vi "Handle Command.vi"(8 "error in (no error)":errorcluster, 9 "Data":variant, 10 "Command":string, 11 "Instrument.Lockin":refnum<class "Instrument.Lockin.lvclass">) -> (0 "error out":errorcluster, 1 "Processed Data":variant, 2 "Command":string, 3 "Instrument.Lockin out":refnum<class "Instrument.Lockin.lvclass">)   [LabVIEW 2019, in "Instrument.Lockin.lvlib" / "Instrument.Lockin.lvclass"]
uses:
  Instrument.Lockin.lvclass
  Typedefs/API/Lockin.Commands.Local--Enum.ctl
  Typedefs/API/Lockin.Commands--Enum.ctl
  Instrument.Lockin.lvclass/Instrument.Lockin.ctl
  <userlib>/LevyLab/Instrument Framework/Instrument Types/Lockin/Typedefs/LockinAPI.Sampling.Sampling--Cluster.ctl
  <userlib>/LevyLab/Instrument Framework/Instrument Types/Lockin/Typedefs/LockinAPI.Sampling.FsMode--enum.ctl
  <userlib>/LevyLab/Instrument Framework/Instrument Types/Lockin/Typedefs/LockinAPI.getState.states--enum.ctl
  <userlib>/LevyLab/Instrument Framework/Instrument Types/Lockin/Typedefs/LockinAPI.SweepData--Cluster.ctl
  Typedefs/API/Lockin.setState--cluster.ctl
  Instrument.DAQ/Typedefs/State--enum.ctl
  Typedefs/API/Lockin.setLogMode--cluster.ctl
  Typedefs/API/Lockin.setAO_Amp--cluster.ctl
  Typedefs/API/Lockin.setAO_DC--cluster.ctl
  Typedefs/API/Lockin.setAO_f--cluster.ctl
  Typedefs/API/Lockin.setAO_phi--cluster.ctl
  Typedefs/API/Lockin.setAO_function--cluster.ctl
  Instrument.DAQ/Typedefs/AO.Channel.Function--Enum.ctl
  Instrument.DAQ/Typedefs/AO.Channel--Cluster--Array.ctl
  Instrument.DAQ/Typedefs/AO.Channel--Cluster.ctl
  Typedefs/API/Lockin.setREF_f--cluster.ctl
  Typedefs/REF Parameter--Enum.ctl
  Typedefs/API/Lockin.setREF_phi--cluster.ctl
  Typedefs/API/Lockin.setREF_TC--cluster.ctl
  Typedefs/API/Lockin.setREF_RollOff--cluster.ctl
  Instrument.DAQ/Typedefs/REF.Channel--Cluster--Array.ctl
  Instrument.DAQ/Typedefs/REF.Channel--Cluster.ctl
  Instrument.DAQ/Typedefs/Sweep.Configuration--Cluster.ctl
  Instrument.DAQ/Typedefs/Sweep.Channel--Cluster--Array.ctl
  Instrument.DAQ/Typedefs/Sweep.Channel--Cluster.ctl
  Instrument.DAQ/Typedefs/Sweep.Pattern--Enum.ctl
  Typedefs/API/Lockin.setSweep_Time--cluster.ctl
  Typedefs/API/Lockin.setSweep_Table--cluster.ctl
  Instrument.DAQ/Typedefs/DAQ.Sampling.Sampling--Cluster.ctl
  Typedefs/API/Lockin.setSamplingFsMode--cluster.ctl
  Instrument.DAQ/Typedefs/DAQ.Sampling.Fs Mode--enum.ctl
  Instrument.DAQ/Typedefs/Channel.Gain--Cluster.ctl
  Instrument.DAQ/Typedefs/DAQ.Configuration--Cluster--Array.ctl
  Instrument.DAQ/Typedefs/DAQ.Configuration--Cluster.ctl
  Instrument.DAQ/Typedefs/DAQ.Config.AO.Range--enum.ctl
  Instrument.DAQ/Typedefs/DAQ.TerminalConfiguration--ring.ctl
  Instrument.DAQ/Typedefs/DAQ.Config.AI.Range--enum.ctl
  Instrument.DAQ/Typedefs/DAQ.Config.AI.Coupling--enum.ctl
  Instrument.DAQ/Typedefs/PrivateEvents--DAQ.showUI.ctl
  Instrument.DAQ/Typedefs/AI.Channel--Cluster--Array.ctl
  Instrument.DAQ/Typedefs/AI.Channel--Cluster.ctl
  Instrument.DAQ/Typedefs/Simulation Mode--enum.ctl
  Typedefs/Offset Mode--Enum.ctl
  Instrument.DAQ/Typedefs/PrivateEvents--DAQ.setCalibration.ctl
  Instrument.DAQ/Typedefs/Configuration.Prefilter--Cluster.ctl
  Instrument.DAQ/Typedefs/Configuration.LinkFrequencies--Cluster.ctl
  Instrument.DAQ/Typedefs/Configuration.AmplitudeLimit--Cluster.ctl
  Instrument.DAQ/Typedefs/Configuration.DCLimit--Cluster.ctl
  Instrument.DAQ/Typedefs/Configuration.DutyCycle--Cluster.ctl
  Typedefs/API/Lockin.setSamplingMode--cluster.ctl
  Instrument.DAQ/Typedefs/DAQ.Sampling.Sample Mode--Ring.ctl
  afc408c1-4a47-494c-817e-7b9f9bb33729.vi
  a7ccf487-04bf-437f-bc58-012293c091eb.vi
  06f5bff1-b823-416c-a758-fc672ecfcc99.vi
  029a7bc4-99e9-4f65-b437-c26585c9cd40.vi
  95117756-58c8-4cf5-b4a1-eea4f9571e2f.vi
  d527b0ad-2cbe-40d7-81d2-49d8d0078832.vi
  c6561379-f98d-4793-93aa-fc4f7b6fa2da.vi
  f7b28b50-f868-4d06-8d90-790d331e6843.vi
  3b890341-4124-4342-9d75-403cba162ea7.vi
  efd52b93-d691-4a9b-b54f-f4c6778ec2a4.vi
  1b48001d-6f4c-40ce-9883-2cfdfc5b0066.vi
  2465c698-e437-4a4f-8860-a626a4e5f6de.vi
  451a16e7-7f0f-4872-98b2-f896a68061ac.vi
  ce862ac6-3818-4682-989c-38fcf43d7c0a.vi
  0f1e83ab-c55c-46b9-bca3-9d617c6a026d.vi
  c46d61d8-ad78-4a4f-bd83-bba7d42c3393.vi
  06811b67-d74b-4972-af3b-9250fa170671.vi
  148daf87-aacf-4ea0-9f45-6b19ec731a12.vi
  b666889e-e9d3-40fa-bff7-b740bef29075.vi
  7fa0c9c7-d96f-42eb-b083-8fec20da1e25.vi
  2eef0b96-7480-46b2-a416-598848f5f946.vi
  4baefe16-dd55-4900-a34f-f85402a43af0.vi
  bf5afc16-6b2f-47bd-9035-54b404507785.vi
  df248ea2-cdbc-4a64-a66c-167358fcc18f.vi
  f4b2f717-a3e3-4701-aa1a-36f1ad587562.vi
  cb03029c-6dea-422e-9ff0-c01ba24202a7.vi
  ea7ae40a-427f-4df9-8330-54c2df2a5be0.vi
  d5077292-e533-4b52-a4d7-ebb5f6280e78.vi
  be7fa38f-04e0-4644-9c08-a6c1d8484273.vi
  228c5f99-5a8a-4ac9-8c3f-6c80f04cbb43.vi
  29174cef-b5b4-4b3d-8dd9-d067235044c7.vi
  0557ee3d-f7cd-4618-85ce-94304b7e905c.vi
  d91f965c-decf-4ad0-9779-3bd2f4599088.vi
  d9adaec0-ad08-4a9e-8669-6c491ae292cb.vi
  acd43294-18b9-4ae6-b527-f08772f90be2.vi
  6a1e6d83-5b10-4acb-978a-0f1ae3d31a35.vi
  847e6f07-fde4-45b3-9907-c341240c9864.vi
  b8b9aa39-8fbe-4465-abb6-4b3c602a596b.vi
  <vilib>/JDP Science/JSONtext/JSON text to Variant.vi
  <vilib>/JDP Science/JSONtext/LVClass Serializer/JSONtext LVClass Serializer.lvclass
  <userlib>/LevyLab/Instrument Framework/Instrument Types/Lockin/Instrument.LockinAPI.lvclass
  Instrument.DAQ/Instrument.DAQ.lvclass
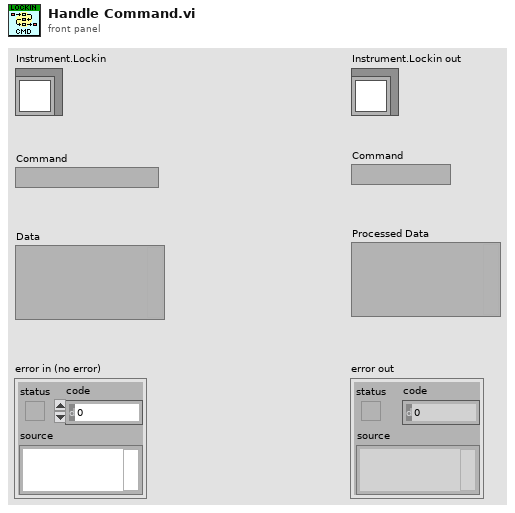
[diagram p1: front panel]
types:
  T1 = typedef "Instrument.Lockin.lvlib/Instrument.Lockin.lvclass/Lockin.Commands.Local--Enum.ctl" = enum16{"autoConfigureDAQ", "setSimulationMode", "zeroPhase", "setCalibration", "setPreFilter", "setFrequencyLink", "setAmplitudeLimit", "setDCLimit", "setDutyCycle", "setSamplingDecimationPreDSP", "setSamplingDecimationPostDSP", "setSamplingMode", "setSamplingFsMultiplier", "setSamplingFsOutput", "setSamplingRefreshRate", "setData_State", "setData_DAQ", "setData_Sampling", "setData_Waveforms", "setData_Results", "setData_SweepWaveforms", "setData_AIChannels", "setData_AOChannels", "setData_REFChannels", "setData_InputGain", "setData_OutputGain", "showUI", "setAI", "setOffset", "setOffsetMode"}
  T2 = typedef "Instrument.Lockin.lvlib/Instrument.Lockin.lvclass/Lockin.Commands--Enum.ctl" = enum16{"setAO", "setAO_Amplitude", "setAO_DC", "setAO_Frequency", "setAO_Phase", "setAO_Function", "setREF", "setREF_Frequency", "setREF_Phase", "setREF_TC", "setREF_Roll-Off", "setDAQ", "setSampling", "setState", "getState", "getAO", "getAI", "getResults", "getSampling", "getAOconfig", "getREFconfig", "setInputGain", "setOutputGain", "getInputGain", "getOutputGain", "setSamplingFsMode", "getSamplingFsMode", "setSweep", "setSweep_Time", "setSweep_Table", "getStatus", "getSweepResults", "getSweepWaveforms", "logConfiguration", "startLogging", "stopLogging"}
  T3 = typedef "Instrument.LockinAPI.lvclass/LockinAPI.Sampling.Sampling--Cluster.ctl" = cluster{"Fs":dbl, "#s":i32}
  T4 = typedef "Instrument.LockinAPI.lvclass/LockinAPI.getState.states--enum.ctl" = enum16{"idle", "created", "started", "stopped", "sweeping"}
  T5 = typedef "Instrument.LockinAPI.lvclass/LockinAPI.SweepData--Cluster.ctl" = cluster{"AO":waveform(dbl)[], "AI":waveform(dbl)[], "X":waveform(dbl)[], "Y":waveform(dbl)[]}
  T6 = cluster{"Time Stamp":timestamp, "Results (Dictionary)":cluster{"key":string, "value":dbl}[]}
  T7 = typedef "Instrument.Lockin.lvlib/Instrument.Lockin.lvclass/Lockin.setState--cluster.ctl" = cluster{"State":T8}
  T8 = typedef "Instrument.Lockin.lvlib/Instrument.DAQ.lvclass/State--enum.ctl" = enum16{"start", "stop", "reset", "start sweep", "stop sweep"}
  T9 = typedef "Instrument.Lockin.lvlib/Instrument.Lockin.lvclass/Lockin.setLogMode--cluster.ctl" = cluster{"interval":u32}
  T10 = enum16{"Amplitude", "DC", "Frequency", "Phase", "Function"}
  T11 = typedef "Instrument.Lockin.lvlib/Instrument.Lockin.lvclass/Lockin.setAO_Amp--cluster.ctl" = cluster{"Channel":i32, "Amplitude":dbl}
  T12 = typedef "Instrument.Lockin.lvlib/Instrument.Lockin.lvclass/Lockin.setAO_DC--cluster.ctl" = cluster{"Channel":i32, "DC":dbl}
  T13 = typedef "Instrument.Lockin.lvlib/Instrument.Lockin.lvclass/Lockin.setAO_f--cluster.ctl" = cluster{"Channel":i32, "Frequency":dbl}
  T14 = typedef "Instrument.Lockin.lvlib/Instrument.Lockin.lvclass/Lockin.setAO_phi--cluster.ctl" = cluster{"Channel":i32, "Phase":dbl}
  T15 = typedef "Instrument.Lockin.lvlib/Instrument.Lockin.lvclass/Lockin.setAO_function--cluster.ctl" = cluster{"Channel":i32, "Function":T16}
  T16 = typedef "Instrument.Lockin.lvlib/Instrument.DAQ.lvclass/AO.Channel.Function--Enum.ctl" = enum16{"sine", "square", "triangle", "saw"}
  T17 = typedef "Instrument.Lockin.lvlib/Instrument.DAQ.lvclass/AO.Channel--Cluster--Array.ctl" = T18[]
  T18 = typedef "Instrument.Lockin.lvlib/Instrument.DAQ.lvclass/AO.Channel--Cluster.ctl" = cluster{"Enable?":bool, "Channel":i32, "Amplitude":dbl, "Offset":dbl, "Frequency":dbl, "Phase":dbl, "Function":T16, "Sweeping?":bool, "Limit AC":bool, "Limit DC?":bool, "Duty Cycle":bool}
  T19 = typedef "Instrument.Lockin.lvlib/Instrument.Lockin.lvclass/Lockin.setREF_f--cluster.ctl" = cluster{"Channel":i32, "Frequency":dbl}
  T20 = typedef "Instrument.Lockin.lvlib/Instrument.Lockin.lvclass/REF Parameter--Enum.ctl" = enum16{"Frequency", "Phase", "Time Constant", "RollOff"}
  T21 = typedef "Instrument.Lockin.lvlib/Instrument.Lockin.lvclass/Lockin.setREF_phi--cluster.ctl" = cluster{"Channel":i32, "Phase":dbl}
  T22 = typedef "Instrument.Lockin.lvlib/Instrument.Lockin.lvclass/Lockin.setREF_TC--cluster.ctl" = cluster{"Channel":i32, "TC":dbl}
  T23 = typedef "Instrument.Lockin.lvlib/Instrument.Lockin.lvclass/Lockin.setREF_RollOff--cluster.ctl" = cluster{"Channel":i32, "Roll-Off":i32}
  T24 = typedef "Instrument.Lockin.lvlib/Instrument.DAQ.lvclass/REF.Channel--Cluster--Array.ctl" = T25[]
  T25 = typedef "Instrument.Lockin.lvlib/Instrument.DAQ.lvclass/REF.Channel--Cluster.ctl" = cluster{"Enable?":bool, "Channel":i32, "Frequency":dbl, "Phase":dbl, "TC":dbl, "Roll-Off":i32}
  T26 = typedef "Instrument.Lockin.lvlib/Instrument.Lockin.lvclass/Lockin.setSweep_Time--cluster.ctl" = cluster{"SweepTime":dbl}
  T27 = typedef "Instrument.Lockin.lvlib/Instrument.Lockin.lvclass/Lockin.setSweep_Table--cluster.ctl" = cluster{"Channel":i32, "Table":dbl[]}
  T28 = typedef "Instrument.Lockin.lvlib/Instrument.DAQ.lvclass/DAQ.Sampling.Sampling--Cluster.ctl" = cluster{"Fs":dbl, "#s":i32}
  T29 = typedef "Instrument.Lockin.lvlib/Instrument.Lockin.lvclass/Lockin.setSamplingFsMode--cluster.ctl" = cluster{"FsMode":T30}
  T30 = typedef "Instrument.Lockin.lvlib/Instrument.DAQ.lvclass/DAQ.Sampling.Fs Mode--enum.ctl" = enum16{"Manual", "Auto Fs", "Max Fs"}
  T31 = typedef "Instrument.Lockin.lvlib/Instrument.DAQ.lvclass/Channel.Gain--Cluster.ctl" = cluster{"Channel":string, "Gain":dbl}
  T32 = typedef "Instrument.Lockin.lvlib/Instrument.DAQ.lvclass/DAQ.Configuration--Cluster--Array.ctl" = T33[]
  T33 = typedef "Instrument.Lockin.lvlib/Instrument.DAQ.lvclass/DAQ.Configuration--Cluster.ctl" = cluster{"Device":string, "Lockin.AO":string, "AO.Ch":string, "AO.Range":T34, "AO terminal config":T35, "Lockin.AI":string, "AI.Ch":string, "AI.Range":T36, "AI.Coupling":T37, "AI terminal config":T35}
  T34 = typedef "Instrument.Lockin.lvlib/Instrument.DAQ.lvclass/DAQ.Config.AO.Range--enum.ctl" = enum16{"±0.1", "±1.0", "±3.5", "±10.0", ""}
  T35 = typedef "Instrument.Lockin.lvlib/Instrument.DAQ.lvclass/DAQ.TerminalConfiguration--ring.ctl" = i32
  T36 = typedef "Instrument.Lockin.lvlib/Instrument.DAQ.lvclass/DAQ.Config.AI.Range--enum.ctl" = enum16{"±0.316", "±1.00", "±3.16", "±10.0", "±31.6", "±42.4", ""}
  T37 = typedef "Instrument.Lockin.lvlib/Instrument.DAQ.lvclass/DAQ.Config.AI.Coupling--enum.ctl" = u16
  T38 = typedef "Instrument.Lockin.lvlib/Instrument.DAQ.lvclass/PrivateEvents--DAQ.showUI.ctl" = bool
  T39 = typedef "Instrument.Lockin.lvlib/Instrument.DAQ.lvclass/AI.Channel--Cluster--Array.ctl" = T40[]
  T40 = typedef "Instrument.Lockin.lvlib/Instrument.DAQ.lvclass/AI.Channel--Cluster.ctl" = cluster{"Enable?":bool, "Channel":i32, "References":u16[], "reference index":i32}
  T41 = typedef "Instrument.Lockin.lvlib/Instrument.DAQ.lvclass/Simulation Mode--enum.ctl" = enum16{"AI = HW simulated", "AI = noise*AO", "AI = waveguide"}
  T42 = typedef "Instrument.Lockin.lvlib/Instrument.Lockin.lvclass/Offset Mode--Enum.ctl" = enum16{"Measure", "Remove"}
  T43 = typedef "Instrument.Lockin.lvlib/Instrument.DAQ.lvclass/PrivateEvents--DAQ.setCalibration.ctl" = enum16{"Check", "Calibrate"}
  T44 = typedef "Instrument.Lockin.lvlib/Instrument.DAQ.lvclass/Configuration.Prefilter--Cluster.ctl" = cluster{"60 Hz":bool, "Low Pass":bool, "Low Pass Cutoff (Hz)":dbl}
  T45 = typedef "Instrument.Lockin.lvlib/Instrument.DAQ.lvclass/Configuration.LinkFrequencies--Cluster.ctl" = cluster{"Link?":bool, "Frequency (Hz)":dbl}
  T46 = typedef "Instrument.Lockin.lvlib/Instrument.DAQ.lvclass/Configuration.DCLimit--Cluster.ctl" = cluster{"Limit?":bool, "Limit (V)":dbl}
  T47 = typedef "Instrument.Lockin.lvlib/Instrument.DAQ.lvclass/Configuration.DutyCycle--Cluster.ctl" = cluster{"Option?":bool, "Duty Cycle (%)":dbl}
  T48 = typedef "Instrument.Lockin.lvlib/Instrument.Lockin.lvclass/Lockin.setSamplingMode--cluster.ctl" = cluster{"SampleMode":T49}
  T49 = typedef "Instrument.Lockin.lvlib/Instrument.DAQ.lvclass/DAQ.Sampling.Sample Mode--Ring.ctl" = i32
  T50 = typedef "Instrument.LockinAPI.lvclass/LockinAPI.Sampling.FsMode--enum.ctl" = enum16{"Manual", "Auto Fs", "Max Fs"}
  T51 = typedef "Instrument.Lockin.lvlib/Instrument.DAQ.lvclass/Status--enum.ctl" = enum16{"idle", "created", "started", "stopped", "sweeping"}
  T52 = typedef "Instrument.Lockin.lvlib/Instrument.DAQ.lvclass/Channel.Gain--Cluster--Array.ctl" = T31[]
  T53 = typedef "Instrument.Lockin.lvlib/Instrument.DAQ.lvclass/Results--Cluster.ctl" = cluster{"Time Stamp":timestamp, "Results (Dictionary)":cluster{"key":string, "value":dbl[]}[]}
  T54 = typedef "Instrument.Lockin.lvlib/Instrument.DAQ.lvclass/Sweep.Configuration--Cluster.ctl" = cluster{"sweepTime":dbl, "initialWaitTime":dbl, "returnToStart":bool, "sweepChannels":T55}
  T55 = typedef "Instrument.Lockin.lvlib/Instrument.DAQ.lvclass/Sweep.Channel--Cluster--Array.ctl" = T56[]
  T56 = typedef "Instrument.Lockin.lvlib/Instrument.DAQ.lvclass/Sweep.Channel--Cluster.ctl" = cluster{"Enable?":bool, "Channel":u16, "Start":dbl, "End":dbl, "Pattern":T57, "Table":dbl[]}
  T57 = typedef "Instrument.Lockin.lvlib/Instrument.DAQ.lvclass/Sweep.Pattern--Enum.ctl" = enum16{"Ramp /", "Ramp /\\", "Smooth Ramp _/", "Smooth Ramp _/\\_", "Table"}
  T58 = typedef "Instrument.Lockin.lvlib/Instrument.DAQ.lvclass/DAQ.Sampling--Cluster.ctl" = cluster{"Sampling":T28, "sample mode":i32, "Fs Mode":T30, "Fs Multiplier":dbl, "Refresh Rate (Hz)":dbl, "Decimation.PreDSP":i32, "Decimation.PostDSP":i32, "Fs.Output":dbl}
  T59 = typedef "Instrument.Lockin.lvlib/Instrument.DAQ.lvclass/DAQ.Config.AO--Cluster--Array.ctl" = cluster{"Channels":tag, "Range":T34, "terminal configuration":T35, "Type":T60}[]
  T60 = typedef "Instrument.Lockin.lvlib/Instrument.DAQ.lvclass/DAQ.Type--enum.ctl" = enum16{"None", "USB-4431", "PXI-446x"}
  T61 = typedef "Instrument.Lockin.lvlib/Instrument.DAQ.lvclass/DAQ.Config.AI--Cluster--Array.ctl" = cluster{"Channels":tag, "Coupling":T37, "Range":T36, "terminal configuration":T35, "Type":T60}[]
  T62 = typedef "Instrument.Lockin.lvlib/Instrument.DAQ.lvclass/PublicEvents--DAQ.getWaveforms.ctl" = cluster{"AO":waveform(dbl)[], "AI":waveform(dbl)[], "REF_X":waveform(dbl)[], "REF_Y":waveform(dbl)[], "X":waveform(dbl)[], "Y":waveform(dbl)[]}
  T63 = typedef "Instrument.Lockin.lvlib/Instrument.DAQ.lvclass/PublicEvents--DAQ.getSweepWaveforms.ctl" = cluster{"AO":waveform(dbl)[], "AI":waveform(dbl)[], "X":waveform(dbl)[], "Y":waveform(dbl)[]}
  T64 = typedef "Instrument.Lockin.lvlib/Instrument.DAQ.lvclass/Configuration.AmplitudeLimit--Cluster.ctl" = cluster{"Limit?":bool, "Limit (V)":dbl}
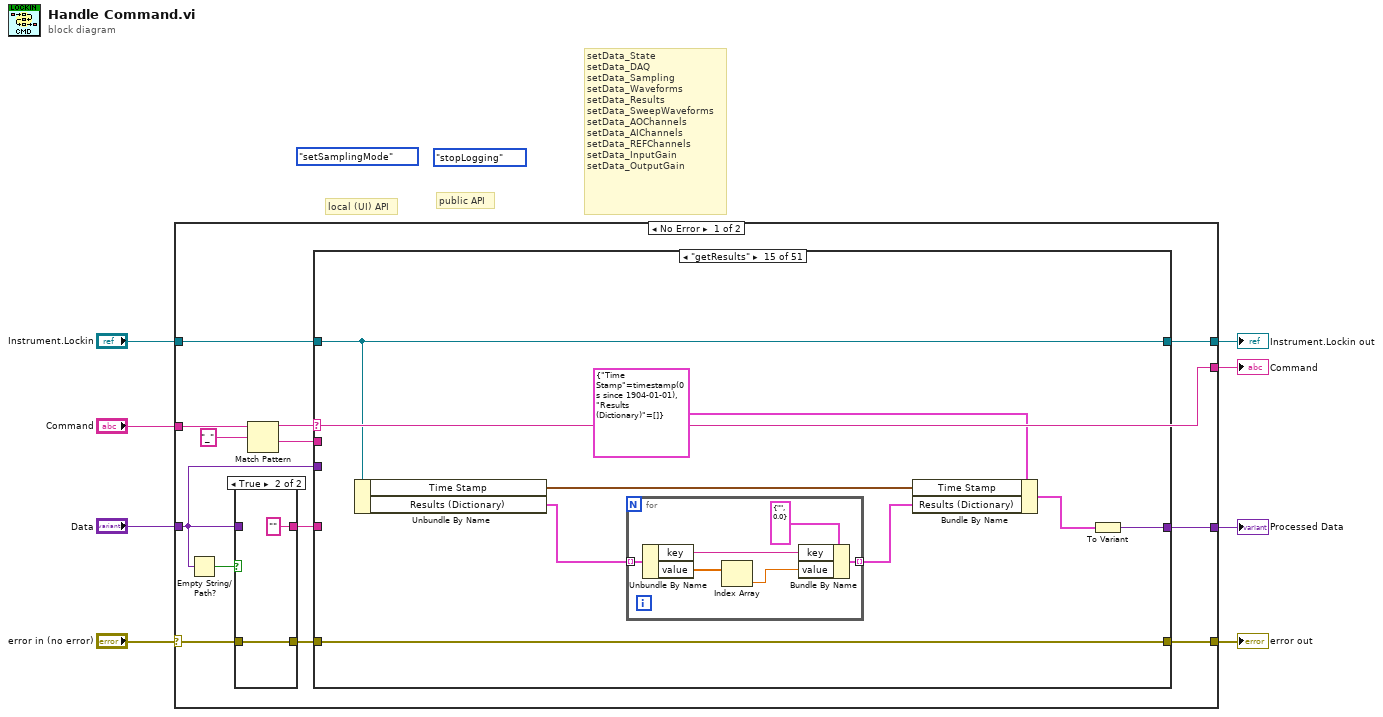
[diagram p0: block diagram]
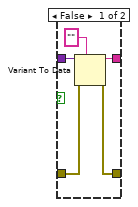
[diagram p2: hidden frame]
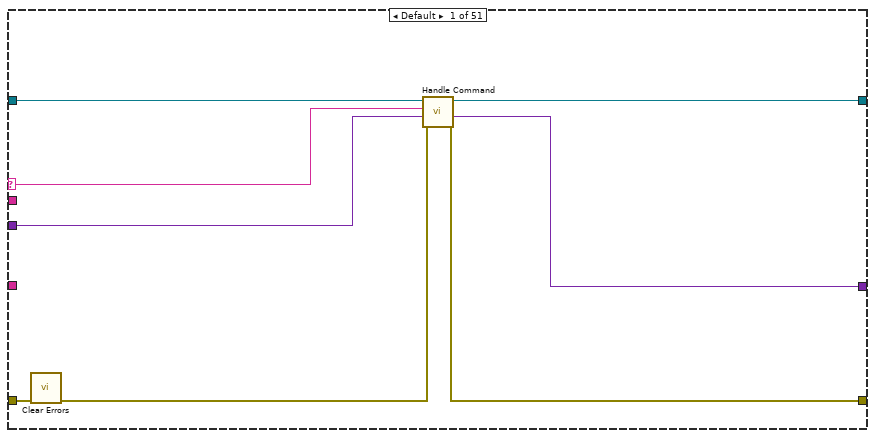
[diagram p3: hidden frame]
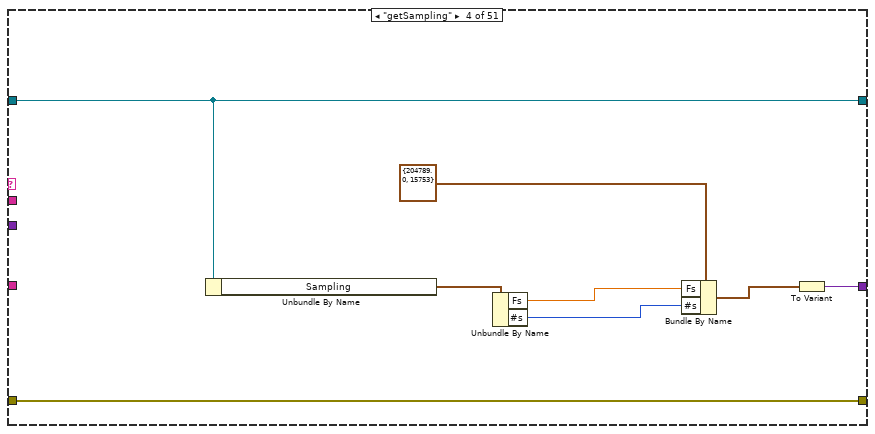
[diagram p6: hidden frame]
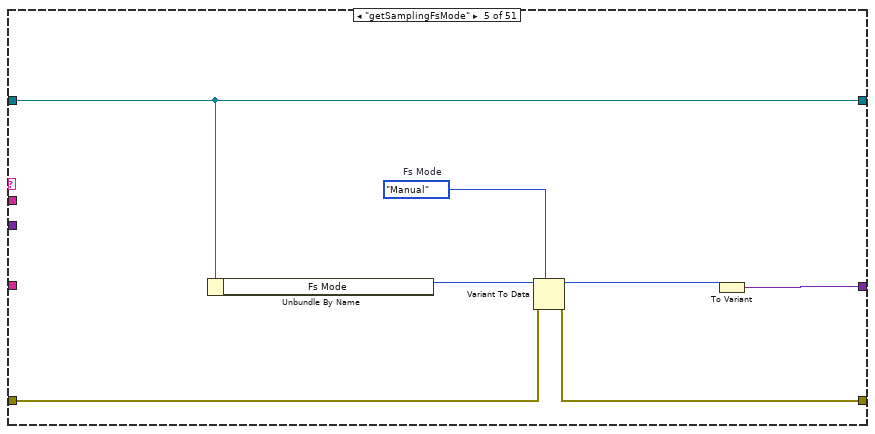
[diagram p7: hidden frame]
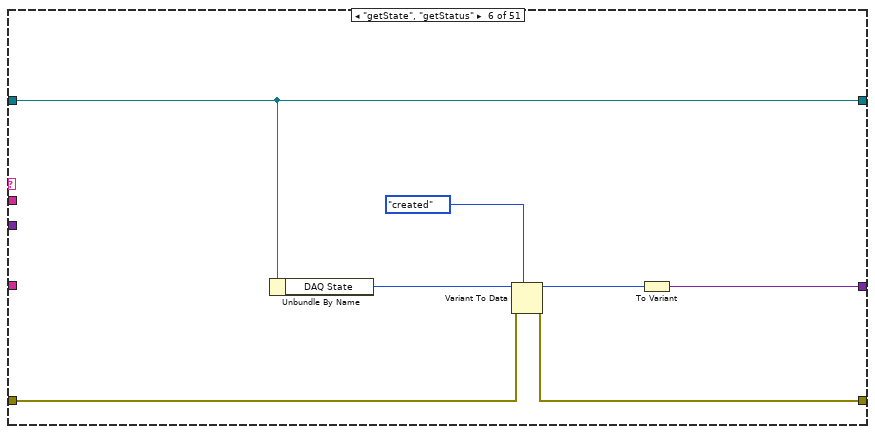
[diagram p8: hidden frame]
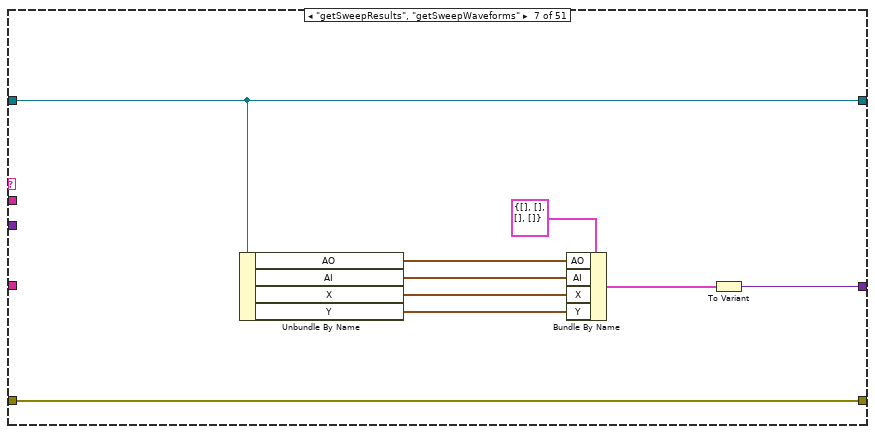
[diagram p9: hidden frame]
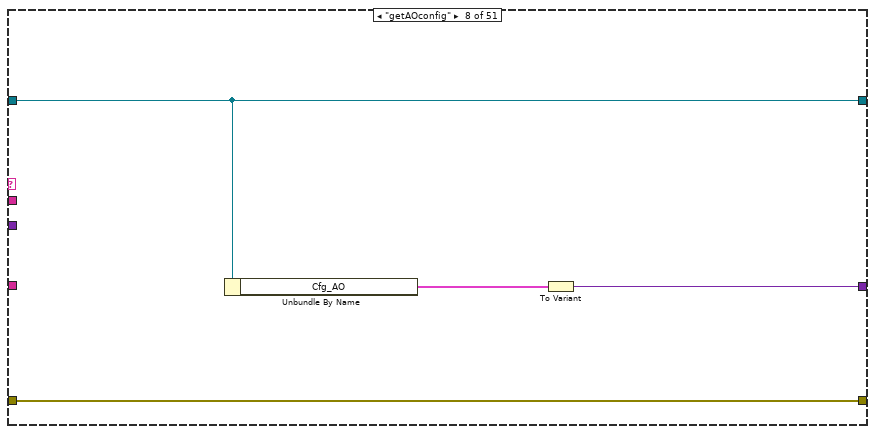
[diagram p10: hidden frame]
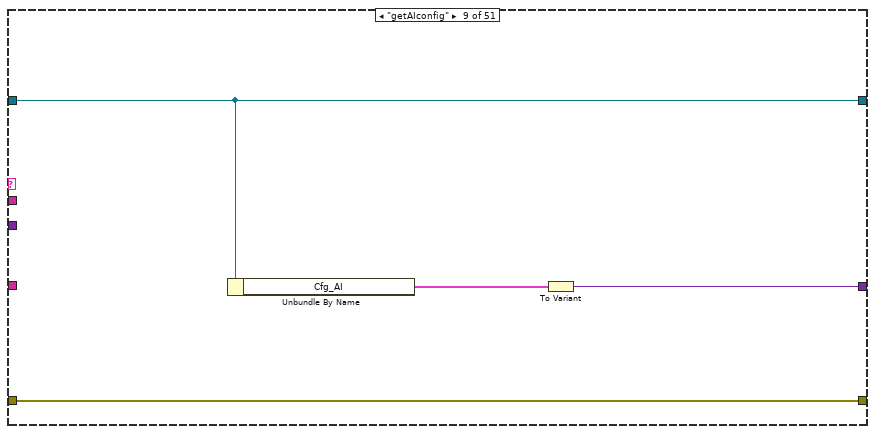
[diagram p11: hidden frame]
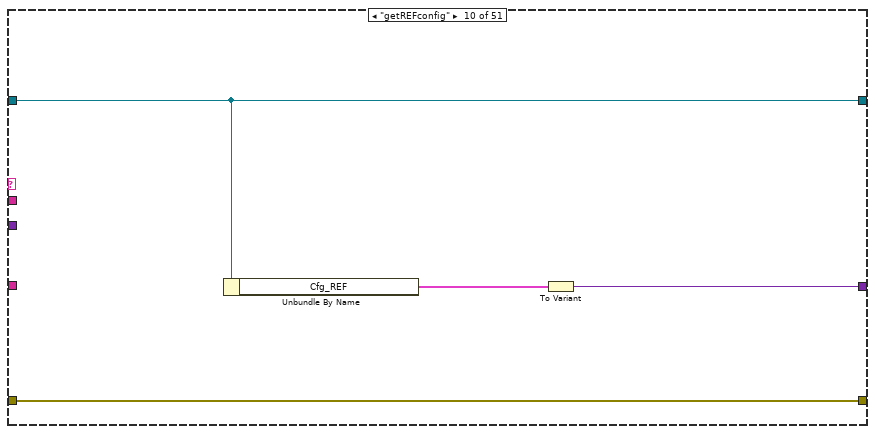
[diagram p12: hidden frame]
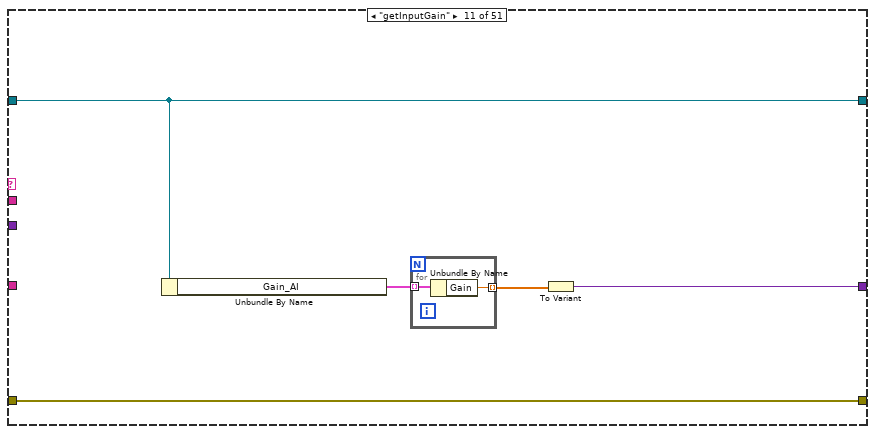
[diagram p13: hidden frame]
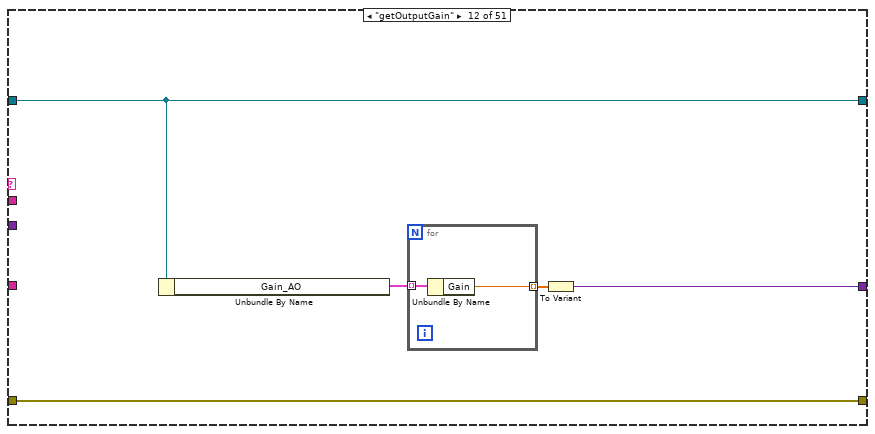
[diagram p14: hidden frame]
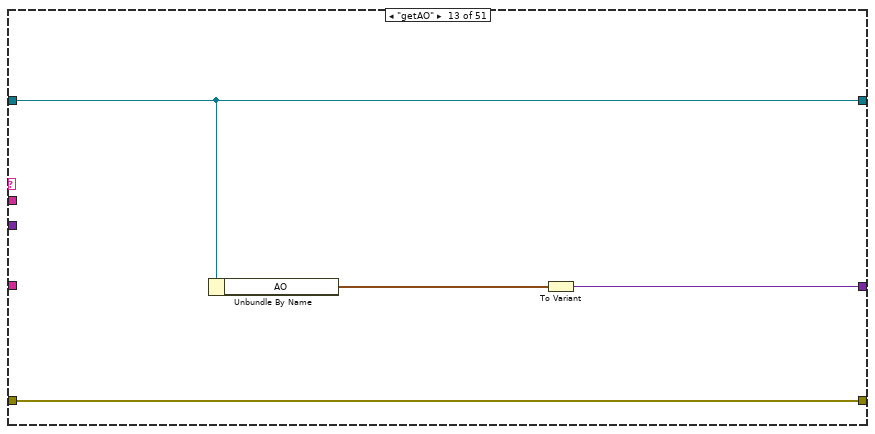
[diagram p15: hidden frame]
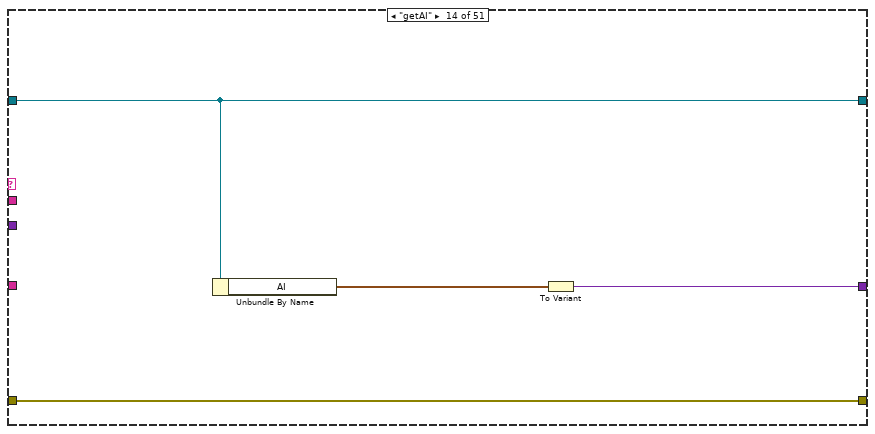
[diagram p16: hidden frame]
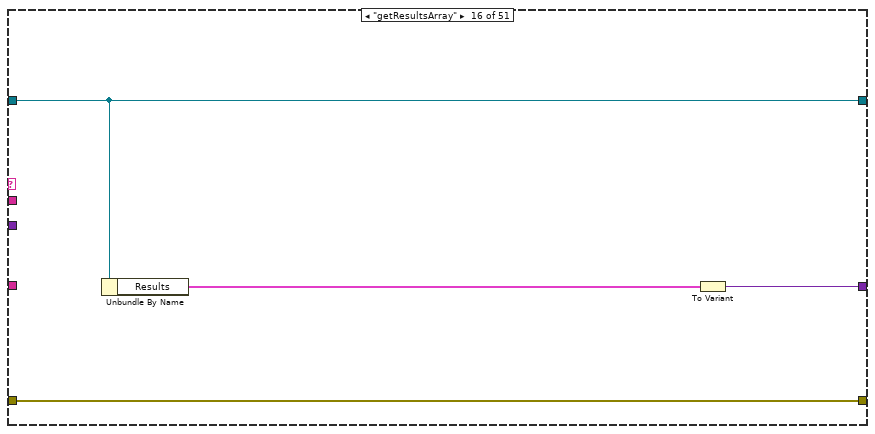
[diagram p17: hidden frame]
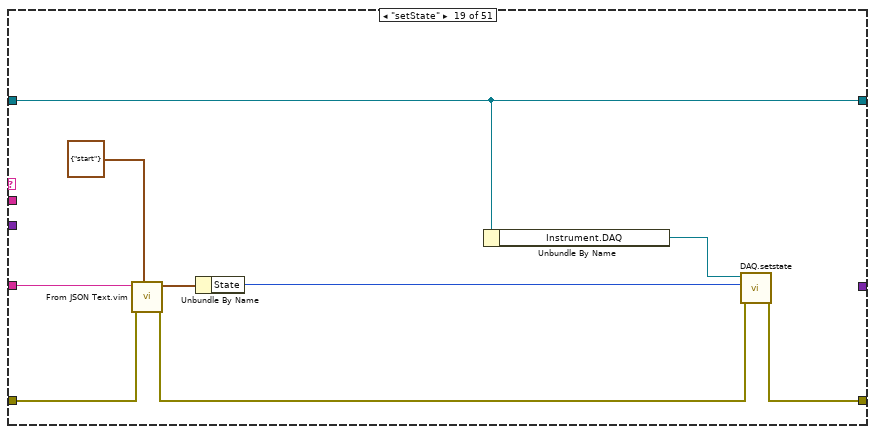
[diagram p20: hidden frame]
diagram:
  (unwired) Lockin.Commands.Local--Enum."setSamplingMode" ("Enum")
  (unwired) Lockin.Commands--Enum."stopLogging" ("Enum")
  # "setData_State\nsetData_DAQ\nsetData_Sampling\nsetData_Waveforms\nsetData_Results\nsetData_SweepWaveforms\nsetData_AOChannels\nsetData_AIChannels\nsetData_REFChannels\nsetData_InputGain\nsetData_OutputGain"
  # "local (UI) API"
  # "public API"
  n1 = case shown="No Error" "error in (no error)" {
    selector: "error in (no error)" -> [w17 w708]
    tunnel: [w18 w708] -> w7
    tunnel: [w20 w707] -> w6
    tunnel: "Instrument.Lockin" -> [w21 w707]
    tunnel: "Command" -> [w12 w706]
    tunnel: [w19 variant] -> w5
    tunnel: "Data" -> [w9 _]
    tunnel: [w11 w706] -> w3
    frame No Error {
      n2 = Empty String/Path?(string/path=w9) -> (empty?=w10:bool)
      n3 = case shown="True" w10 {
        tunnel: w17 -> [w26 w27]
        tunnel: [w24 ""] -> w16
        tunnel: [w23 w27] -> w13
        tunnel: w9 -> [w22 _]
        frame False {
          n4 = Variant To Data(error in=w26, type="", Variant=w22) -> (data=w24:string, error out=w23:errorcluster)
        }
        frame True {
        }
      }
      n5 = Match Pattern(string=w12, regular expression="_") -> (before substring=w11:string, after substring=w14:string)  [unwired: 1 in, 2 out]
      n6 = case shown="\"getResults\"" w11 {
        selector: w11 -> [w31 _ _ _ _ _ _ _ _ _ _ _ _ _ _ _ _ _ _ _ _ _ _ _ _ _ _ _ _ _ _ _ _ _ _ _ _ _ _ _ _ _ _ _ _ _ _ _ _ _ _]
        tunnel: w21 -> [w36 w38 w40 w46 w54 w61 w69 w72 w76 w80 w86 w93 w98 w102 w111 w121 w125 w127 w131 w140 w147 w151 w156 w230 w293 w325 w340 w349 w367 w386 w403 w414 w416 w430 w438 w552 w565 w575 w585 w593 w600 w612 w622 w632 w642 w650 w660 w674 w684 w694 w704]
        tunnel: [w34 w38 w40 w46 w54 w61 w69 w72 w76 w80 w86 w93 w98 w102 w111 w121 w125 w127 w131 w140 w147 w151 w154 w225 w297 w324 w337 w350 w368 w387 w402 w414 w416 w424 w434 w552 w564 w575 w585 w593 w601 w613 w623 w633 w643 w649 w659 w671 w681 w691 w701] -> w20
        tunnel: [w35 _ _ w48 w55 w62 w71 w74 w78 w82 w88 w95 w101 w105 w113 w123 _ _ _ _ _ _ _ _ _ _ _ _ _ _ _ _ _ _ _ _ _ w566 _ _ _ _ _ _ _ _ _ _ _ _ _] -> w19
        tunnel: w16 -> [_ _ _ _ _ _ _ _ _ _ _ _ _ _ _ _ _ _ w136 w144 _ _ w160 w233 w301 w331 w342 w355 w373 w391 w412 _ w422 w432 w436 _ w559 w572 _ w590 w597 w608 w618 w631 w641 w648 w658 w669 w678 w688 w699]
        tunnel: [w32 w37 w39 w47 w50 w57 w70 w73 w77 w81 w87 w94 w100 w104 w112 w122 w124 w126 w132 w137 w146 w150 w157 w226 w298 w327 w335 w351 w369 w388 w407 w413 w417 w426 w433 w554 w560 w573 w583 w591 w602 w609 w619 w625 w634 w651 w661 w670 w680 w690 w700] -> w18
        tunnel: w14 -> [_ _ _ _ _ _ _ _ _ _ _ _ _ _ _ _ _ _ _ _ _ _ w155 w231 w294 _ _ _ _ _ _ _ _ _ w437 _ _ _ _ _ _ _ _ _ _ _ _ _ _ _ _]
        tunnel: w13 -> [w33 w37 w39 w47 w49 w56 w70 w73 w77 w81 w87 w94 w100 w104 w112 w122 w124 w126 w135 w143 w145 w148 w159 w232 w300 w329 w341 w354 w372 w390 w411 w413 w419 w431 w435 w553 w558 w569 w584 w586 w595 w606 w615 w629 w639 w647 w657 w668 w676 w687 w696]
        tunnel: w9 -> [w30 _ _ _ _ _ _ _ _ _ _ _ _ _ _ _ _ _ _ _ _ _ _ _ _ _ _ _ _ _ _ _ _ _ _ _ _ _ _ _ _ _ _ _ _ _ _ _ _ _ _]
        frame Default {
          n7 = call <vilib>:"Clear Errors.vi"("error in (no error)"=w33) -> ("error out"=w29:errorcluster)  [unwired: 5 in, 1 out]
          n8 = call-parent "Handle Command.vi"("error in (no error)"=w29, "params in"=w30, "command"=w31, "Instrument in"=w36) -> ("error out"=w32:errorcluster, "processed data"=w35:variant, "Instrument out"=w34:refnum<class "Instrument.Lockin.lvclass">)  [unwired: 4 in, 1 out]
        }
        frame "----------PUBLIC API----------" {
        }
        frame "----------GET METHODS----------" {
        }
        frame "getSampling" {
          n9 = Unbundle By Name(w46) -> ("Sampling"=w44:T28)
          n10 = Unbundle By Name(w44) -> ("Fs"=w43:dbl, "#s"=w42:i32)
          n11 = Bundle By Name(cluster=T3 {"Fs"=204789.0, "#s"=15753} ("sampling"), "Fs"=w43, "#s"=w42) -> (w41:T3)
          n12 = To Variant(anything=w41) -> (Variant=w48:variant)
        }
        frame "getSamplingFsMode" {
          w52 = LockinAPI.Sampling.FsMode--enum."Manual"  # Fs Mode
          n13 = Unbundle By Name(w54) -> ("Fs Mode"=w53:T30)
          n14 = Variant To Data(error in=w49, type=w52, Variant=w53) -> (data=w51:T50, error out=w50:errorcluster)
          n15 = To Variant(anything=w51) -> (Variant=w55:variant)
        }
        frame "getState", "getStatus" {
          n16 = Unbundle By Name(w61) -> ("DAQ State"=w59:T51)
          n17 = Variant To Data(error in=w56, type=LockinAPI.getState.states--enum."created" ("getState.states"), Variant=w59) -> (data=w58:T4, error out=w57:errorcluster)
          n18 = To Variant(anything=w58) -> (Variant=w62:variant)
        }
        frame "getSweepResults", "getSweepWaveforms" {
          n19 = Unbundle By Name(w69) -> ("AO"=w67:waveform(dbl)[], "AI"=w66:waveform(dbl)[], "X"=w65:waveform(dbl)[], "Y"=w64:waveform(dbl)[])
          n20 = Bundle By Name(cluster=T5 {"AO"=[], "AI"=[], "X"=[], "Y"=[]} ("sweepData"), "AO"=w67, "AI"=w66, "X"=w65, "Y"=w64) -> (w63:T5)
          n21 = To Variant(anything=w63) -> (Variant=w71:variant)
        }
        frame "getAOconfig" {
          n22 = Unbundle By Name(w72) -> ("Cfg_AO"=w75:T17)
          n23 = To Variant(anything=w75) -> (Variant=w74:variant)
        }
        frame "getAIconfig" {
          n24 = Unbundle By Name(w76) -> ("Cfg_AI"=w79:T39)
          n25 = To Variant(anything=w79) -> (Variant=w78:variant)
        }
        frame "getREFconfig" {
          n26 = Unbundle By Name(w80) -> ("Cfg_REF"=w83:T24)
          n27 = To Variant(anything=w83) -> (Variant=w82:variant)
        }
        frame "getInputGain" {
          n28 = Unbundle By Name(w86) -> ("Gain_AI"=w85:T52)
          n29 = for {
            tunnel: w85 -> [w90] mode=indexing
            tunnel: [w89] -> w84 mode=indexing
            n30 = Unbundle By Name(w90) -> ("Gain"=w89:dbl)
          }
          n31 = To Variant(anything=w84) -> (Variant=w88:variant)
        }
        frame "getOutputGain" {
          n32 = Unbundle By Name(w93) -> ("Gain_AO"=w92:T52)
          n33 = for {
            tunnel: w92 -> [w97] mode=indexing
            tunnel: [w96] -> w91 mode=indexing
            n34 = Unbundle By Name(w97) -> ("Gain"=w96:dbl)
          }
          n35 = To Variant(anything=w91) -> (Variant=w95:variant)
        }
        frame "getAO" {
          n36 = Unbundle By Name(w98) -> ("AO"=w99:waveform(dbl)[])
          n37 = To Variant(anything=w99) -> (Variant=w101:variant)
        }
        frame "getAI" {
          n38 = Unbundle By Name(w102) -> ("AI"=w103:waveform(dbl)[])
          n39 = To Variant(anything=w103) -> (Variant=w105:variant)
        }
        frame "getResults" {
          n40 = Unbundle By Name(w111) -> ("Time Stamp"=w108:timestamp, "Results (Dictionary)"=w107:cluster{"key":string, "value":dbl[]}[])
          n41 = for {
            tunnel: w107 -> [w118] mode=indexing
            tunnel: [w114] -> w109 mode=indexing
            n42 = Unbundle By Name(w118) -> ("key"=w115:string, "value"=w119:dbl[])
            n43 = Index Array(array=w119) -> (element=w116:dbl)  [unwired: 1 in]
            n44 = Bundle By Name(cluster=cluster{"key":string, "value":dbl} {"key"="", "value"=0.0} ("key-value"), "key"=w115, "value"=w116) -> (w114:cluster{"key":string, "value":dbl})
          }
          n45 = Bundle By Name(cluster=T6 {"Time Stamp"=timestamp(0 s since 1904-01-01), "Results (Dictionary)"=[]} ("input cluster"), "Time Stamp"=w108, "Results (Dictionary)"=w109) -> (w106:T6)
          n46 = To Variant(anything=w106) -> (Variant=w113:variant)
        }
        frame "getResultsArray" {
          n47 = Unbundle By Name(w121) -> ("Results"=w120:T53)
          n48 = To Variant(anything=w120) -> (Variant=w123:variant)
        }
        frame "getAUX" {
        }
        frame "----------SET METHODS----------" {
        }
        frame "setState" {
          n49 = call "From JSON Text.vim"("Data Type and Default Value"=T7 {"State"=enum."start"} ("setState"), "error in (no error)"=w135, "JSON"=w136) -> ("error out"=w133:errorcluster, "Data out"=w129:T7)  [unwired: 7 in]
          n50 = Unbundle By Name(w129) -> ("State"=w128:T8)
          n51 = Unbundle By Name(w131) -> ("Instrument.DAQ"=w134:refnum<class "Instrument.DAQ.lvclass">)
          n52 = call "DAQ.setstate.vi"("error in (no error)"=w133, "setState"=w128, "Instrument.DAQ"=w134) -> ("error out"=w132:errorcluster)  [unwired: 7 in, 1 out]
        }
        frame "startLogging" {
          # "local event API does not need cluster"
          # "remote API store data in cluster"
          n53 = call "From JSON Text.vim"("Data Type and Default Value"=T9 {"interval"=1} ("setLogMode"), "error in (no error)"=w143, "JSON"=w144) -> ("error out"=w138:errorcluster, "Data out"=w142:T9)  [unwired: 7 in]
          n54 = Unbundle By Name(w142) -> ("interval"=w139:u32)
          n55 = call "Lockin.setLogMode.vi"("error in (no error)"=w138, "interval (ms)"=w139, "Instrument.Lockin"=w140) -> ("error out"=w137:errorcluster)  [unwired: 7 in, 1 out]
        }
        frame "logConfiguration" {
          # "local event API does not need cluster"
          # "remote API store data in cluster"
          n56 = call "Lockin.logConfiguration.vi"("error in (no error)"=w145, "Instrument.Lockin"=w147) -> ("error out"=w146:errorcluster)  [unwired: 8 in, 1 out]
        }
        frame "stopLogging" {
          # "local event API does not need cluster"
          n57 = call "Lockin.setLogMode.vi"("error in (no error)"=w148, "interval (ms)"=u32 0 ("interval"), "Instrument.Lockin"=w151) -> ("error out"=w150:errorcluster)  [unwired: 7 in, 1 out]
        }
        frame "setAO" {
          # "Lockin SMO: Set AO"
          # "Adjust Channels"
          n58 = case shown="\"\"" w155 {
            selector: w155 -> [w170 _]
            tunnel: w160 -> [w169 w222]
            tunnel: w159 -> [w168 w221]
            tunnel: [w163 w217] -> w153
            tunnel: w156 -> [w166 w220]
            tunnel: [w167 w219] -> w154
            frame Default {
              n59 = case shown="\"Phase\"" w170 {
                tunnel: w169 -> [w179 w188 w197 w206 w215]
                tunnel: w168 -> [w178 w187 w196 w205 w214]
                tunnel: [w177 w186 w195 w204 w213] -> w164
                tunnel: [T10."Amplitude" ("Parameter") T10."DC" ("Parameter") T10."Frequency" ("Parameter") T10."Phase" ("Parameter") T10."Function" ("Parameter")] -> w165
                tunnel: [w173 w183 w192 w201 w210] -> w162
                tunnel: [w171 w180 w189 w198 w207] -> w161
                frame "Amplitude", Default {
                  n60 = call "From JSON Text.vim"("Data Type and Default Value"=T11 {"Channel"=5, "Amplitude"=0.0} ("setAO_Amp"), "error in (no error)"=w178, "JSON"=w179) -> ("error out"=w177:errorcluster, "Data out"=w175:T11)  [unwired: 7 in]
                  n61 = Unbundle By Name(w175) -> ("Channel"=w173:i32, "Amplitude"=w172:dbl)
                  n62 = To Variant(anything=w172) -> (Variant=w171:variant)
                }
                frame "DC" {
                  n63 = call "From JSON Text.vim"("Data Type and Default Value"=T12 {"Channel"=5, "DC"=0.0} ("setAO_DC"), "error in (no error)"=w187, "JSON"=w188) -> ("error out"=w186:errorcluster, "Data out"=w185:T12)  [unwired: 7 in]
                  n64 = Unbundle By Name(w185) -> ("Channel"=w183:i32, "DC"=w182:dbl)
                  n65 = To Variant(anything=w182) -> (Variant=w180:variant)
                }
                frame "Frequency" {
                  n66 = call "From JSON Text.vim"("Data Type and Default Value"=T13 {"Channel"=5, "Frequency"=0.0} ("setAO_f"), "error in (no error)"=w196, "JSON"=w197) -> ("error out"=w195:errorcluster, "Data out"=w194:T13)  [unwired: 7 in]
                  n67 = Unbundle By Name(w194) -> ("Channel"=w192:i32, "Frequency"=w191:dbl)
                  n68 = To Variant(anything=w191) -> (Variant=w189:variant)
                }
                frame "Phase" {
                  n69 = call "From JSON Text.vim"("Data Type and Default Value"=T14 {"Channel"=5, "Phase"=0.0} ("setAO_phi"), "error in (no error)"=w205, "JSON"=w206) -> ("error out"=w204:errorcluster, "Data out"=w203:T14)  [unwired: 7 in]
                  n70 = Unbundle By Name(w203) -> ("Channel"=w201:i32, "Phase"=w200:dbl)
                  n71 = To Variant(anything=w200) -> (Variant=w198:variant)
                }
                frame "Function" {
                  n72 = call "From JSON Text.vim"("Data Type and Default Value"=T15 {"Channel"=5, "Function"=enum."sine"} ("setAO_function"), "error in (no error)"=w214, "JSON"=w215) -> ("error out"=w213:errorcluster, "Data out"=w212:T15)  [unwired: 7 in]
                  n73 = Unbundle By Name(w212) -> ("Channel"=w210:i32, "Function"=w209:T16)
                  n74 = To Variant(anything=w209) -> (Variant=w207:variant)
                }
              }
              n75 = call "Update AO Parameter.vi"("Parameter"=w165, "error in"=w164, "Value"=w161, "Channel"=w162, "Instrument.Lockin"=w166) -> ("error out"=w163:errorcluster, "Instrument.Lockin out"=w167:refnum<class "Instrument.Lockin.lvclass">)  [unwired: 5 in]
            }
            frame "" {
              n76 = call "From JSON Text.vim"("Data Type and Default Value"=T17 [] ("AO Channels"), "error in (no error)"=w221, "JSON"=w222) -> ("error out"=w217:errorcluster, "Data out"=w218:T17)  [unwired: 7 in]
              n77 = Bundle By Name(cluster=w220, "Cfg_AO"=w218) -> (w219:refnum<class "Instrument.Lockin.lvclass">)
            }
          }
          n78 = Unbundle By Name(w154) -> ("Instrument.DAQ"=w158:refnum<class "Instrument.DAQ.lvclass">, "Cfg_AO"=w152:T17)
          n79 = call "DAQ.setAO.vi"("error in (no error)"=w153, "AO Channels"=w152, "Instrument.DAQ"=w158) -> ("error out"=w157:errorcluster)  [unwired: 7 in, 1 out]
        }
        frame "setREF" {
          # "Lockin SMO: Set REF"
          # "Adjust Channels"
          n80 = case shown="Default" w231 {
            selector: w231 -> [w247 _]
            tunnel: w233 -> [w246 w290]
            tunnel: w232 -> [w245 w289]
            tunnel: [w242 w285] -> w224
            tunnel: w230 -> [w244 w288]
            tunnel: [w243 w287] -> w225
            frame Default {
              n81 = case shown="\"Frequency\", Default" w247 {
                tunnel: w246 -> [w256 w265 w274 w283]
                tunnel: w245 -> [w255 w264 w273 w282]
                tunnel: [w254 w263 w272 w281] -> w240
                tunnel: [REF_Parameter--Enum."Frequency" ("Parameter") REF_Parameter--Enum."Phase" ("Parameter") REF_Parameter--Enum."Time Constant" ("Parameter") REF_Parameter--Enum."RollOff" ("Parameter")] -> w241
                tunnel: [w252 w261 w270 w279] -> w238
                tunnel: [w250 w259 w268 w277] -> w239
                frame "Frequency", Default {
                  n82 = call "From JSON Text.vim"("Data Type and Default Value"=T19 {"Channel"=0, "Frequency"=0.0} ("setREF_f"), "error in (no error)"=w255, "JSON"=w256) -> ("error out"=w254:errorcluster, "Data out"=w253:T19)  [unwired: 7 in]
                  n83 = Unbundle By Name(w253) -> ("Channel"=w252:i32, "Frequency"=w251:dbl)
                  n84 = To Variant(anything=w251) -> (Variant=w250:variant)
                }
                frame "Phase" {
                  n85 = call "From JSON Text.vim"("Data Type and Default Value"=T21 {"Channel"=0, "Phase"=0.0} ("setREF_phi"), "error in (no error)"=w264, "JSON"=w265) -> ("error out"=w263:errorcluster, "Data out"=w262:T21)  [unwired: 7 in]
                  n86 = Unbundle By Name(w262) -> ("Channel"=w261:i32, "Phase"=w260:dbl)
                  n87 = To Variant(anything=w260) -> (Variant=w259:variant)
                }
                frame "TC" {
                  n88 = call "From JSON Text.vim"("Data Type and Default Value"=T22 {"Channel"=0, "TC"=1e-05} ("setREF_phi"), "error in (no error)"=w273, "JSON"=w274) -> ("error out"=w272:errorcluster, "Data out"=w271:T22)  [unwired: 7 in]
                  n89 = Unbundle By Name(w271) -> ("Channel"=w270:i32, "TC"=w269:dbl)
                  n90 = To Variant(anything=w269) -> (Variant=w268:variant)
                }
                frame "RollOff" {
                  n91 = call "From JSON Text.vim"("Data Type and Default Value"=T23 {"Channel"=0, "Roll-Off"=1} ("setREF_Roll-Off"), "error in (no error)"=w282, "JSON"=w283) -> ("error out"=w281:errorcluster, "Data out"=w280:T23)  [unwired: 7 in]
                  n92 = Unbundle By Name(w280) -> ("Channel"=w279:i32, "Roll-Off"=w278:i32)
                  n93 = To Variant(anything=w278) -> (Variant=w277:variant)
                }
              }
              n94 = call "Update REF Parameter.vi"("Parameter"=w241, "error in"=w240, "Value"=w239, "Channel"=w238, "Instrument.Lockin"=w244) -> ("error out"=w242:errorcluster, "Instrument.Lockin out"=w243:refnum<class "Instrument.Lockin.lvclass">)  [unwired: 5 in]
            }
            frame "" {
              n95 = call "From JSON Text.vim"("Data Type and Default Value"=T24 [] ("REF Channels"), "error in (no error)"=w289, "JSON"=w290) -> ("error out"=w285:errorcluster, "Data out"=w286:T24)  [unwired: 7 in]
              n96 = Bundle By Name(cluster=w288, "Cfg_REF"=w286) -> (w287:refnum<class "Instrument.Lockin.lvclass">)
            }
          }
          n97 = Unbundle By Name(w225) -> ("Instrument.DAQ"=w229:refnum<class "Instrument.DAQ.lvclass">, "Cfg_REF"=w223:T24)
          n98 = call "DAQ.setREF.vi"("error in (no error)"=w224, "Channels: Lockin"=w223, "Instrument.DAQ"=w229) -> ("error out"=w227:errorcluster, "Instrument.DAQ out"=w228:refnum<class "Instrument.DAQ.lvclass">)  [unwired: 7 in]
          n99 = disable-structure shown="Disabled" {
            disable-tunnel: w228 -> [w236 _]
            disable-tunnel: w227 -> [w235 w237]
            disable-tunnel: [w234 w237] -> w226
            frame Disabled {
              # "Lockin SMO: Reset Phase"
              n100 = call "DAQ.zeroPhase.vi"("error in (no error)"=w235, "Instrument.DAQ"=w236) -> ("error out"=w234:errorcluster)  [unwired: 8 in, 1 out]
            }
            frame Enabled {
            }
          }
        }
        frame "setSweep" {
          n101 = Unbundle By Name(w293) -> ("Sweep"=w292:T54)
          n102 = case shown="\"Time\"" w294 {
            tunnel: w301 -> [w305 w314 w321]
            tunnel: w300 -> [w304 w313 w320]
            tunnel: [w303 w312 w319] -> w299
            tunnel: [w302 w308 w317] -> w291
            tunnel: w292 -> [_ w310 w318]
            frame "", Default {
              w306 = T54 {"sweepTime"=0.0, "initialWaitTime"=0.0, "returnToStart"=FALSE, "sweepChannels"=[]}  # Configure Sweep
              n103 = call "From JSON Text.vim"("Data Type and Default Value"=w306, "error in (no error)"=w304, "JSON"=w305) -> ("error out"=w303:errorcluster, "Data out"=w302:T54)  [unwired: 7 in]
            }
            frame "Time" {
              n104 = call "From JSON Text.vim"("Data Type and Default Value"=T26 {"SweepTime"=0.0} ("setSweep_Time"), "error in (no error)"=w313, "JSON"=w314) -> ("error out"=w312:errorcluster, "Data out"=w309:T26)  [unwired: 7 in]
              n105 = Unbundle By Name(w309) -> ("SweepTime"=w307:dbl)
              n106 = Bundle By Name(cluster=w310, "sweepTime"=w307) -> (w308:T54)
            }
            frame "Table" {
              n107 = call "From JSON Text.vim"("Data Type and Default Value"=T27[] [] ("Array"), "error in (no error)"=w320, "JSON"=w321) -> ("error out"=w319:errorcluster, "Data out"=w315:T27[])  [unwired: 7 in]
              n108 = call "Replace Sweep Waveforms.vi"("Channels New"=w315, "Sweep in"=w318) -> ("Sweep out"=w317:T54)  [unwired: 9 in]
            }
          }
          n109 = Bundle By Name(cluster=w293, "Sweep"=w291) -> (w297:refnum<class "Instrument.Lockin.lvclass">)
          n110 = Unbundle By Name(w297) -> ("Instrument.DAQ"=w296:refnum<class "Instrument.DAQ.lvclass">, "Sweep"=w295:T54)
          n111 = call "DAQ.setSweep.vi"("error in (no error)"=w299, "setSweep"=w295, "Instrument.DAQ"=w296) -> ("error out"=w298:errorcluster)  [unwired: 7 in, 1 out]
        }
        frame "setSampling" {
          n112 = call "From JSON Text.vim"("Data Type and Default Value"=T28 {"Fs"=204789.0, "#s"=15753}, "error in (no error)"=w329, "JSON"=w331) -> ("error out"=w322:errorcluster, "Data out"=w323:T28)  [unwired: 7 in]
          n113 = Bundle By Name(cluster=w325, "Sampling"=w323) -> (w324:refnum<class "Instrument.Lockin.lvclass">)
          n114 = Unbundle By Name(w324) -> ("Instrument.DAQ"=w328:refnum<class "Instrument.DAQ.lvclass">, "Sampling"=w326:T58)
          n115 = call "DAQ.setSampling.vi"("error in (no error)"=w322, "Sampling"=w326, "Instrument.DAQ"=w328) -> ("error out"=w327:errorcluster)  [unwired: 7 in, 1 out]
        }
        frame "setSamplingFsMode" {
          n116 = call "From JSON Text.vim"("Data Type and Default Value"=T29 {"FsMode"=enum."Manual"} ("setSampleFsMode"), "error in (no error)"=w341, "JSON"=w342) -> ("error out"=w336:errorcluster, "Data out"=w334:T29)  [unwired: 7 in]
          n117 = Unbundle By Name(w334) -> ("FsMode"=w333:T30)
          n118 = Bundle By Name(cluster=w340, "Fs Mode"=w333) -> (w337:refnum<class "Instrument.Lockin.lvclass">)
          n119 = Unbundle By Name(w337) -> ("Instrument.DAQ"=w339:refnum<class "Instrument.DAQ.lvclass">, "Sampling"=w338:T58)
          n120 = call "DAQ.setSampling.vi"("error in (no error)"=w336, "Sampling"=w338, "Instrument.DAQ"=w339) -> ("error out"=w335:errorcluster)  [unwired: 7 in, 1 out]
        }
        frame "setInputGain" {
          n121 = call "From JSON Text.vim"("Data Type and Default Value"=dbl[] [], "error in (no error)"=w354, "JSON"=w355) -> ("error out"=w353:errorcluster, "Data out"=w346:dbl[])  [unwired: 7 in]
          n122 = for {
            tunnel: T31 {"Channel"="AI1", "Gain"=1.0} ("System Cluster") -> [w360]
            tunnel: w346 -> [w359] mode=indexing
            tunnel: [w358] -> w345 mode=indexing
            n123 = Bundle By Name(cluster=w360, "Gain"=w359) -> (w358:T31)
          }
          n124 = Bundle By Name(cluster=w349, "Gain_AI"=w345) -> (w350:refnum<class "Instrument.Lockin.lvclass">)
          n125 = Unbundle By Name(w350) -> ("Instrument.DAQ"=w352:refnum<class "Instrument.DAQ.lvclass">, "Gain_AI"=w344:T52)
          n126 = for {
            tunnel: w344 -> [w357] mode=indexing
            tunnel: [w356] -> w343 mode=indexing
            n127 = Unbundle By Name(w357) -> ("Gain"=w356:dbl)
          }
          n128 = call "DAQ.setInputGain.vi"("error in (no error)"=w353, "Input Gain"=w343, "Instrument.DAQ"=w352) -> ("error out"=w351:errorcluster)  [unwired: 7 in, 1 out]
        }
        frame "setOffset" {
          n129 = call "From JSON Text.vim"("Data Type and Default Value"=dbl[] [], "error in (no error)"=w372, "JSON"=w373) -> ("error out"=w371:errorcluster, "Data out"=w364:dbl[])  [unwired: 7 in]
          n130 = for {
            tunnel: T31 {"Channel"="AI1", "Gain"=1.0} ("System Cluster") -> [w378]
            tunnel: w364 -> [w377] mode=indexing
            tunnel: [w376] -> w363 mode=indexing
            n131 = Bundle By Name(cluster=w378, "Gain"=w377) -> (w376:T31)
          }
          n132 = Bundle By Name(cluster=w367, "Offset_AI"=w363) -> (w368:refnum<class "Instrument.Lockin.lvclass">)
          n133 = Unbundle By Name(w368) -> ("Instrument.DAQ"=w370:refnum<class "Instrument.DAQ.lvclass">, "Offset_AI"=w362:T52)
          n134 = for {
            tunnel: w362 -> [w375] mode=indexing
            tunnel: [w374] -> w361 mode=indexing
            n135 = Unbundle By Name(w375) -> ("Gain"=w374:dbl)
          }
          n136 = call "DAQ.setInputOffset.vi"("error in (no error)"=w371, "Input Offset"=w361, "Instrument.DAQ"=w370) -> ("error out"=w369:errorcluster)  [unwired: 7 in, 1 out]
        }
        frame "setOutputGain" {
          n137 = call "From JSON Text.vim"("Data Type and Default Value"=dbl[] [], "error in (no error)"=w390, "JSON"=w391) -> ("error out"=w385:errorcluster, "Data out"=w382:dbl[])  [unwired: 7 in]
          n138 = for {
            tunnel: T31 {"Channel"="AI1", "Gain"=1.0} ("System Cluster") -> [w396]
            tunnel: w382 -> [w395] mode=indexing
            tunnel: [w394] -> w381 mode=indexing
            n139 = Bundle By Name(cluster=w396, "Gain"=w395) -> (w394:T31)
          }
          n140 = Bundle By Name(cluster=w386, "Gain_AO"=w381) -> (w387:refnum<class "Instrument.Lockin.lvclass">)
          n141 = Unbundle By Name(w387) -> ("Instrument.DAQ"=w389:refnum<class "Instrument.DAQ.lvclass">, "Gain_AO"=w380:T52)
          n142 = for {
            tunnel: w380 -> [w393] mode=indexing
            tunnel: [w392] -> w379 mode=indexing
            n143 = Unbundle By Name(w393) -> ("Gain"=w392:dbl)
          }
          n144 = call "DAQ.setOutputGain.vi"("error in (no error)"=w385, "Output Gain"=w379, "Instrument.DAQ"=w389) -> ("error out"=w388:errorcluster)  [unwired: 7 in, 1 out]
        }
        frame "setDAQ" {
          n145 = call "From JSON Text.vim"("Data Type and Default Value"=T32 [] ("DAQ.Config []"), "error in (no error)"=w411, "JSON"=w412) -> ("error out"=w401:errorcluster, "Data out"=w409:T32)  [unwired: 7 in]
          n146 = call "config UI to not UI (AO and AI).vi"("New Ch []"=w409) -> ("AO Config"=w398:T59, "AI Config"=w397:T61)  [unwired: 9 in]
          n147 = Bundle By Name(cluster=w403, "AI"=w397, "AO"=w398) -> (w402:refnum<class "Instrument.Lockin.lvclass">)
          n148 = Unbundle By Name(w402) -> ("Instrument.DAQ"=w404:refnum<class "Instrument.DAQ.lvclass">, "AI"=w406:T61, "Simulation mode"=w399:T41, "AO"=w405:T59)
          n149 = call "DAQ.setAIconfig.vi"("error in (no error)"=w401, "Simulation mode"=w399, "AI Configuration"=w406, "Instrument.DAQ"=w404) -> ("error out"=w408:errorcluster, "Instrument.DAQ out"=w410:refnum<class "Instrument.DAQ.lvclass">)  [unwired: 6 in]
          n150 = call "DAQ.setAOconfig.vi"("error in (no error)"=w408, "AO Configuration"=w405, "Instrument.DAQ"=w410) -> ("error out"=w407:errorcluster)  [unwired: 7 in, 1 out]
        }
        frame "----------LOCAL API----------" {
        }
        frame "showUI" {
          n151 = call "From JSON Text.vim"("Data Type and Default Value"=T38 FALSE ("show UI?"), "error in (no error)"=w419, "JSON"=w422) -> ("error out"=w418:errorcluster, "Data out"=w420:T38)  [unwired: 7 in]
          n152 = Unbundle By Name(w416) -> ("Instrument.DAQ"=w415:refnum<class "Instrument.DAQ.lvclass">)
          n153 = call "DAQ.showUI.vi"("error in (no error)"=w418, "show UI?"=w420, "Instrument.DAQ"=w415) -> ("error out"=w417:errorcluster)  [unwired: 7 in, 1 out]
        }
        frame "setAI" {
          # "Lockin SMO: Set AI"
          n154 = call "From JSON Text.vim"("Data Type and Default Value"=T39 [] ("AI Channels"), "error in (no error)"=w431, "JSON"=w432) -> ("error out"=w425:errorcluster, "Data out"=w423:T39)  [unwired: 7 in]
          n155 = Bundle By Name(cluster=w430, "Cfg_AI"=w423) -> (w424:refnum<class "Instrument.Lockin.lvclass">)
          n156 = Unbundle By Name(w424) -> ("Instrument.DAQ"=w428:refnum<class "Instrument.DAQ.lvclass">, "Cfg_AI"=w427:T39)
          n157 = call "DAQ.setAI.vi"("error in (no error)"=w425, "AI Channels"=w427, "Instrument.DAQ"=w428) -> ("error out"=w426:errorcluster)  [unwired: 7 in, 1 out]
        }
        frame "setData" {
          n158 = case shown="\"OutputGain\"" w437 {
            tunnel: w438 -> [w440 w449 w460 w469 w471 w483 w495 w514 w523 w532 w541 w550]
            tunnel: w436 -> [_ w446 w455 w466 w474 w486 w497 w510 w520 w525 w538 w547]
            tunnel: w435 -> [w439 w442 w454 w465 w473 w485 w498 w509 w518 w529 w537 w546]
            tunnel: [w440 w448 w459 w468 w470 w482 w494 w513 w522 w531 w540 w549] -> w434
            tunnel: [w439 w444 w452 w463 w472 w484 w496 w507 w516 w527 w535 w544] -> w433
            frame Default {
            }
            frame "State" {
              n159 = Unbundle By Name(w449) -> ("DAQ State"=w441:T51)
              n160 = Unflatten From String(type=w441, binary string=w446, error in (no error)=w442) -> (value=w447:T51, error out=w445:errorcluster)  [unwired: 2 in, 1 out]
              n161 = Variant To Data(error in=w445, type=w441, Variant=w447) -> (data=w443:T51, error out=w444:errorcluster)
              n162 = Bundle By Name(cluster=w449, "DAQ State"=w443) -> (w448:refnum<class "Instrument.Lockin.lvclass">)
            }
            frame "DAQ" {
              w450 = T32 [] ("DAQ.Config []")
              # "only setData is flatten to string. otherwise use JSON"
              n163 = Unflatten From String(type=w450, binary string=w455, error in (no error)=w454) -> (value=w456:T32, error out=w453:errorcluster)  [unwired: 2 in, 1 out]
              n164 = Variant To Data(error in=w453, type=w450, Variant=w456) -> (data=w451:T32, error out=w452:errorcluster)
              n165 = call "config UI to not UI (AO and AI).vi"("New Ch []"=w451) -> ("AO Config"=w458:T59, "AI Config"=w457:T61)  [unwired: 9 in]
              n166 = Bundle By Name(cluster=w460, "AI"=w457, "AO"=w458) -> (w459:refnum<class "Instrument.Lockin.lvclass">)
            }
            frame "Sampling" {
              n167 = Unbundle By Name(w469) -> ("Sampling"=w461:T58)
              n168 = Unflatten From String(type=w461, binary string=w466, error in (no error)=w465) -> (value=w467:T58, error out=w464:errorcluster)  [unwired: 2 in, 1 out]
              n169 = Variant To Data(error in=w464, type=w461, Variant=w467) -> (data=w462:T58, error out=w463:errorcluster)
              n170 = Bundle By Name(cluster=w469, "Sampling"=w462) -> (w468:refnum<class "Instrument.Lockin.lvclass">)
            }
            frame "Waveforms" {
              n171 = in-place {
                in-place-border: w474 -> [w480]
                in-place-border: w473 -> [w479]
                in-place-border: [w477] -> w472
                n172 = in-place-cluster #1(w471) -> ("Waveforms"=w476:T62)
                n173 = Unflatten From String(type=w476, binary string=w480, error in (no error)=w479) -> (value=w481:T62, error out=w478:errorcluster)  [unwired: 2 in, 1 out]
                n174 = Variant To Data(error in=w478, type=w476, Variant=w481) -> (data=w475:T62, error out=w477:errorcluster)
                n175 = in-place-cluster #1("Waveforms"=w475) -> (w470:refnum<class "Instrument.Lockin.lvclass">)
              }
            }
            frame "Results" {
              n176 = in-place {
                in-place-border: w486 -> [w492]
                in-place-border: w485 -> [w491]
                in-place-border: [w489] -> w484
                n177 = in-place-cluster #2(w483) -> ("Results"=w487:T53)
                n178 = Unflatten From String(type=w487, binary string=w492, error in (no error)=w491) -> (value=w493:T53, error out=w490:errorcluster)  [unwired: 2 in, 1 out]
                n179 = Variant To Data(error in=w490, type=w487, Variant=w493) -> (data=w488:T53, error out=w489:errorcluster)
                n180 = in-place-cluster #2("Results"=w488) -> (w482:refnum<class "Instrument.Lockin.lvclass">)
              }
            }
            frame "SweepWaveforms" {
              n181 = in-place {
                in-place-border: w498 -> [w504]
                in-place-border: w497 -> [w503]
                in-place-border: [w501] -> w496
                n182 = in-place-cluster #3(w495) -> ("SweepWaveforms"=w500:T63)
                n183 = Unflatten From String(type=w500, binary string=w503, error in (no error)=w504) -> (value=w505:T63, error out=w502:errorcluster)  [unwired: 2 in, 1 out]
                n184 = Variant To Data(error in=w502, type=w500, Variant=w505) -> (data=w499:T63, error out=w501:errorcluster)
                n185 = in-place-cluster #3("SweepWaveforms"=w499) -> (w494:refnum<class "Instrument.Lockin.lvclass">)
              }
            }
            frame "AOChannels" {
              n186 = Unbundle By Name(w514) -> ("Cfg_AO"=w506:T17)
              n187 = Unflatten From String(type=w506, binary string=w510, error in (no error)=w509) -> (value=w512:T17, error out=w508:errorcluster)  [unwired: 2 in, 1 out]
              n188 = Variant To Data(error in=w508, type=w506, Variant=w512) -> (data=w511:T17, error out=w507:errorcluster)
              n189 = Bundle By Name(cluster=w514, "Cfg_AO"=w511) -> (w513:refnum<class "Instrument.Lockin.lvclass">)
            }
            frame "AIChannels" {
              n190 = Unbundle By Name(w523) -> ("Cfg_AI"=w515:T39)
              n191 = Unflatten From String(type=w515, binary string=w520, error in (no error)=w518) -> (value=w521:T39, error out=w517:errorcluster)  [unwired: 2 in, 1 out]
              n192 = Variant To Data(error in=w517, type=w515, Variant=w521) -> (data=w519:T39, error out=w516:errorcluster)
              n193 = Bundle By Name(cluster=w523, "Cfg_AI"=w519) -> (w522:refnum<class "Instrument.Lockin.lvclass">)
            }
            frame "REFChannels" {
              n194 = Unbundle By Name(w532) -> ("Cfg_REF"=w524:T24)
              n195 = Unflatten From String(type=w524, binary string=w525, error in (no error)=w529) -> (value=w530:T24, error out=w528:errorcluster)  [unwired: 2 in, 1 out]
              n196 = Variant To Data(error in=w528, type=w524, Variant=w530) -> (data=w526:T24, error out=w527:errorcluster)
              n197 = Bundle By Name(cluster=w532, "Cfg_REF"=w526) -> (w531:refnum<class "Instrument.Lockin.lvclass">)
            }
            frame "InputGain" {
              n198 = Unbundle By Name(w541) -> ("Gain_AI"=w533:T52)
              n199 = Unflatten From String(type=w533, binary string=w538, error in (no error)=w537) -> (value=w539:T52, error out=w536:errorcluster)  [unwired: 2 in, 1 out]
              n200 = Variant To Data(error in=w536, type=w533, Variant=w539) -> (data=w534:T52, error out=w535:errorcluster)
              n201 = Bundle By Name(cluster=w541, "Gain_AI"=w534) -> (w540:refnum<class "Instrument.Lockin.lvclass">)
            }
            frame "OutputGain" {
              n202 = Unbundle By Name(w550) -> ("Gain_AO"=w542:T52)
              n203 = Unflatten From String(type=w542, binary string=w547, error in (no error)=w546) -> (value=w548:T52, error out=w545:errorcluster)  [unwired: 2 in, 1 out]
              n204 = Variant To Data(error in=w545, type=w542, Variant=w548) -> (data=w543:T52, error out=w544:errorcluster)
              n205 = Bundle By Name(cluster=w550, "Gain_AO"=w543) -> (w549:refnum<class "Instrument.Lockin.lvclass">)
            }
          }
        }
        frame "autoConfigureDAQ" {
          n206 = Unbundle By Name(w552) -> ("Instrument.DAQ"=w551:refnum<class "Instrument.DAQ.lvclass">)
          n207 = call "DAQ.autoConfigureDAQ.vi"("error in (no error)"=w553, "Instrument.DAQ"=w551) -> ("error out"=w554:errorcluster)  [unwired: 8 in, 1 out]
        }
        frame "setSimulationMode" {
          n208 = call "From JSON Text.vim"("Data Type and Default Value"=Simulation_Mode--enum."AI = noise*AO" ("AI Simulation mode"), "error in (no error)"=w558, "JSON"=w559) -> ("error out"=w557:errorcluster, "Data out"=w555:T41)  [unwired: 7 in]
          n209 = Bundle By Name(cluster=w565, "Simulation mode"=w555) -> (w564:refnum<class "Instrument.Lockin.lvclass">)
          n210 = Unbundle By Name(w564) -> ("Instrument.DAQ"=w563:refnum<class "Instrument.DAQ.lvclass">, "AI"=w562:T61, "Simulation mode"=w561:T41)
          n211 = call "DAQ.setAIconfig.vi"("error in (no error)"=w557, "Simulation mode"=w561, "AI Configuration"=w562, "Instrument.DAQ"=w563) -> ("error out"=w560:errorcluster)  [unwired: 6 in, 1 out]
        }
        frame "setOffsetMode" {
          n212 = Build Array(Offset_Mode--Enum."Remove" ("Offset Mode")) -> (w567:T42[])
          n213 = call "From JSON Text.vim"("Data Type and Default Value"=w567, "error in (no error)"=w569, "JSON"=w572) -> ("error out"=w568:errorcluster, "Data out"=w570:T42[])  [unwired: 7 in]
          n214 = Index Array(array=w570) -> (element=w566:T42)  [unwired: 1 in]
          n215 = Unbundle By Name(w575) -> ("Instrument.DAQ"=w574:refnum<class "Instrument.DAQ.lvclass">)
          n216 = case shown="\"Measure\"" w566 {
            tunnel: w574 -> [w578 w581]
            tunnel: w568 -> [w577 w580]
            tunnel: [w576 w579] -> w573
            frame "Measure" {
              n217 = call "DAQ.measureOffset.vi"("error in (no error)"=w577, "Instrument.DAQ"=w578) -> ("error out"=w576:errorcluster)  [unwired: 8 in, 1 out]
            }
            frame "Remove" {
              n218 = call "DAQ.zeroOffset.vi"("error in (no error)"=w580, "Instrument.DAQ"=w581) -> ("error out"=w579:errorcluster)  [unwired: 8 in, 1 out]
            }
          }
        }
        frame "zeroPhase" {
          n219 = Unbundle By Name(w585) -> ("Instrument.DAQ"=w582:refnum<class "Instrument.DAQ.lvclass">)
          n220 = call "DAQ.zeroPhase.vi"("error in (no error)"=w584, "Instrument.DAQ"=w582) -> ("error out"=w583:errorcluster)  [unwired: 8 in, 1 out]
        }
        frame "setCalibration" {
          n221 = call "From JSON Text.vim"("Data Type and Default Value"=PrivateEvents--DAQ.setCalibration."Check" ("setCalibration"), "error in (no error)"=w586, "JSON"=w590) -> ("error out"=w587:errorcluster, "Data out"=w588:T43)  [unwired: 7 in]
          n222 = Unbundle By Name(w593) -> ("Instrument.DAQ"=w592:refnum<class "Instrument.DAQ.lvclass">)
          n223 = call "DAQ.setCalibration.vi"("error in (no error)"=w587, "setCalibration"=w588, "Instrument.DAQ"=w592) -> ("error out"=w591:errorcluster)  [unwired: 7 in, 1 out]
        }
        frame "setPreFilter" {
          n224 = call "From JSON Text.vim"("Data Type and Default Value"=T44 {"60 Hz"=FALSE, "Low Pass"=FALSE, "Low Pass Cutoff (Hz)"=0.0} ("PreFilter"), "error in (no error)"=w595, "JSON"=w597) -> ("error out"=w594:errorcluster, "Data out"=w596:T44)  [unwired: 7 in]
          n225 = Bundle By Name(cluster=w600, "Prefilter"=w596) -> (w601:refnum<class "Instrument.Lockin.lvclass">)
          n226 = Unbundle By Name(w601) -> ("Instrument.DAQ"=w603:refnum<class "Instrument.DAQ.lvclass">, "Prefilter"=w599:T44)
          n227 = call "DAQ.setPreFilter.vi"("error in (no error)"=w594, "PreFilter"=w599, "Instrument.DAQ"=w603) -> ("error out"=w602:errorcluster)  [unwired: 7 in, 1 out]
        }
        frame "setFrequencyLink" {
          n228 = call "From JSON Text.vim"("Data Type and Default Value"=T45 {"Link?"=FALSE, "Frequency (Hz)"=0.0} ("Link Frequencies"), "error in (no error)"=w606, "JSON"=w608) -> ("error out"=w605:errorcluster, "Data out"=w604:T45)  [unwired: 7 in]
          n229 = Bundle By Name(cluster=w612, "Link Frequencies"=w604) -> (w613:refnum<class "Instrument.Lockin.lvclass">)
          n230 = Unbundle By Name(w613) -> ("Instrument.DAQ"=w611:refnum<class "Instrument.DAQ.lvclass">, "Link Frequencies"=w610:T45)
          n231 = call "DAQ.setLinkFrequencies.vi"("error in (no error)"=w605, "Link Frequencies"=w610, "Instrument.DAQ"=w611) -> ("error out"=w609:errorcluster)  [unwired: 7 in, 1 out]
        }
        frame "setAmplitudeLimit" {
          w617 = T64 {"Limit?"=FALSE, "Limit (V)"=0.0}  # Limit Amplitude
          n232 = call "From JSON Text.vim"("Data Type and Default Value"=w617, "error in (no error)"=w615, "JSON"=w618) -> ("error out"=w614:errorcluster, "Data out"=w616:T64)  [unwired: 7 in]
          n233 = Bundle By Name(cluster=w622, "Amplitude Limit"=w616) -> (w623:refnum<class "Instrument.Lockin.lvclass">)
          n234 = Unbundle By Name(w623) -> ("Instrument.DAQ"=w621:refnum<class "Instrument.DAQ.lvclass">, "Amplitude Limit"=w620:T64)
          n235 = call "DAQ.setAmplitudeLimit.vi"("error in (no error)"=w614, "Amplitude Limit"=w620, "Instrument.DAQ"=w621) -> ("error out"=w619:errorcluster)  [unwired: 7 in, 1 out]
        }
        frame "setDCLimit" {
          n236 = call "From JSON Text.vim"("Data Type and Default Value"=T46 {"Limit?"=FALSE, "Limit (V)"=0.0} ("DC Limit"), "error in (no error)"=w629, "JSON"=w631) -> ("error out"=w626:errorcluster, "Data out"=w630:T46)  [unwired: 7 in]
          n237 = Bundle By Name(cluster=w632, "DC Limit"=w630) -> (w633:refnum<class "Instrument.Lockin.lvclass">)
          n238 = Unbundle By Name(w633) -> ("Instrument.DAQ"=w628:refnum<class "Instrument.DAQ.lvclass">, "DC Limit"=w627:T46)
          n239 = call "DAQ.setDCLimit.vi"("error in (no error)"=w626, "DC Limit"=w627, "Instrument.DAQ"=w628) -> ("error out"=w625:errorcluster)  [unwired: 7 in, 1 out]
        }
        frame "setDutyCycle" {
          n240 = call "From JSON Text.vim"("Data Type and Default Value"=T47 {"Option?"=FALSE, "Duty Cycle (%)"=0.0} ("Function Option"), "error in (no error)"=w639, "JSON"=w641) -> ("error out"=w635:errorcluster, "Data out"=w640:T47)  [unwired: 7 in]
          n241 = Bundle By Name(cluster=w642, "Duty Cycle"=w640) -> (w643:refnum<class "Instrument.Lockin.lvclass">)
          n242 = Unbundle By Name(w643) -> ("Instrument.DAQ"=w637:refnum<class "Instrument.DAQ.lvclass">, "Duty Cycle"=w636:T47)
          n243 = call "DAQ.setDutyCycle.vi"("error in (no error)"=w635, "Duty Cycle"=w636, "Instrument.DAQ"=w637) -> ("error out"=w634:errorcluster)  [unwired: 7 in, 1 out]
        }
        frame "setSamplingDecimationPreDSP" {
          n244 = call "From JSON Text.vim"("Data Type and Default Value"=0, "error in (no error)"=w647, "JSON"=w648) -> ("error out"=w646:errorcluster, "Data out"=w645:i32)  [unwired: 7 in]
          n245 = Bundle By Name(cluster=w650, "Decimation.PreDSP"=w645) -> (w649:refnum<class "Instrument.Lockin.lvclass">)
          n246 = Unbundle By Name(w649) -> ("Instrument.DAQ"=w653:refnum<class "Instrument.DAQ.lvclass">, "Sampling"=w652:T58)
          n247 = call "DAQ.setSampling.vi"("error in (no error)"=w646, "Sampling"=w652, "Instrument.DAQ"=w653) -> ("error out"=w651:errorcluster)  [unwired: 7 in, 1 out]
        }
        frame "setSamplingDecimationPostDSP" {
          n248 = call "From JSON Text.vim"("Data Type and Default Value"=0, "error in (no error)"=w657, "JSON"=w658) -> ("error out"=w656:errorcluster, "Data out"=w655:i32)  [unwired: 7 in]
          n249 = Bundle By Name(cluster=w660, "Decimation.PreDSP"=w655) -> (w659:refnum<class "Instrument.Lockin.lvclass">)
          n250 = Unbundle By Name(w659) -> ("Instrument.DAQ"=w663:refnum<class "Instrument.DAQ.lvclass">, "Sampling"=w662:T58)
          n251 = call "DAQ.setSampling.vi"("error in (no error)"=w656, "Sampling"=w662, "Instrument.DAQ"=w663) -> ("error out"=w661:errorcluster)  [unwired: 7 in, 1 out]
        }
        frame "setSamplingMode" {
          (unwired) DAQ.Sampling.Fs_Mode--enum."Manual"  # Fs Mode
          # "#todo\nAUTO sampling mode"
          n252 = call "From JSON Text.vim"("Data Type and Default Value"=T48 {"SampleMode"=10123} ("setSampleMode"), "error in (no error)"=w668, "JSON"=w669) -> ("error out"=w667:errorcluster, "Data out"=w665:T48)  [unwired: 7 in]
          n253 = Unbundle By Name(w665) -> ("SampleMode"=w664:T49)
          n254 = Bundle By Name(cluster=w674, "sample mode"=w664) -> (w671:refnum<class "Instrument.Lockin.lvclass">)
          n255 = Unbundle By Name(w671) -> ("Instrument.DAQ"=w673:refnum<class "Instrument.DAQ.lvclass">, "Sampling"=w672:T58)
          n256 = call "DAQ.setSampling.vi"("error in (no error)"=w667, "Sampling"=w672, "Instrument.DAQ"=w673) -> ("error out"=w670:errorcluster)  [unwired: 7 in, 1 out]
        }
        frame "setSamplingFsMultiplier" {
          n257 = call "From JSON Text.vim"("Data Type and Default Value"=0.0, "error in (no error)"=w676, "JSON"=w678) -> ("error out"=w675:errorcluster, "Data out"=w677:dbl)  [unwired: 7 in]
          n258 = Bundle By Name(cluster=w684, "Fs Multiplier"=w677) -> (w681:refnum<class "Instrument.Lockin.lvclass">)
          n259 = Unbundle By Name(w681) -> ("Instrument.DAQ"=w683:refnum<class "Instrument.DAQ.lvclass">, "Sampling"=w682:T58)
          n260 = call "DAQ.setSampling.vi"("error in (no error)"=w675, "Sampling"=w682, "Instrument.DAQ"=w683) -> ("error out"=w680:errorcluster)  [unwired: 7 in, 1 out]
        }
        frame "setSamplingFsOutput" {
          n261 = call "From JSON Text.vim"("Data Type and Default Value"=0.0, "error in (no error)"=w687, "JSON"=w688) -> ("error out"=w686:errorcluster, "Data out"=w685:dbl)  [unwired: 7 in]
          n262 = Bundle By Name(cluster=w694, "Fs.Output"=w685) -> (w691:refnum<class "Instrument.Lockin.lvclass">)
          n263 = Unbundle By Name(w691) -> ("Instrument.DAQ"=w693:refnum<class "Instrument.DAQ.lvclass">, "Sampling"=w692:T58)
          n264 = call "DAQ.setSampling.vi"("error in (no error)"=w686, "Sampling"=w692, "Instrument.DAQ"=w693) -> ("error out"=w690:errorcluster)  [unwired: 7 in, 1 out]
        }
        frame "setSamplingRefreshRate" {
          n265 = call "From JSON Text.vim"("Data Type and Default Value"=0.0, "error in (no error)"=w696, "JSON"=w699) -> ("error out"=w695:errorcluster, "Data out"=w697:dbl)  [unwired: 7 in]
          n266 = Bundle By Name(cluster=w704, "Refresh Rate (Hz)"=w697) -> (w701:refnum<class "Instrument.Lockin.lvclass">)
          n267 = Unbundle By Name(w701) -> ("Instrument.DAQ"=w703:refnum<class "Instrument.DAQ.lvclass">, "Sampling"=w702:T58)
          n268 = call "DAQ.setSampling.vi"("error in (no error)"=w695, "Sampling"=w702, "Instrument.DAQ"=w703) -> ("error out"=w700:errorcluster)  [unwired: 7 in, 1 out]
        }
      }
    }
    frame Error {
    }
  }
  "error out" <- w7
  "Instrument.Lockin out" <- w6
  "Command" <- w3
  "Processed Data" <- w5
